vi "CSTK_Icon_Creator_Dialong_InputPath.vi"(0 "Enable":bool=TRUE caption="启用", 1 "分类文件夹名输入":string caption="分类文件夹名", 5 "error in (no error)":errorcluster caption="错误输入（无错误）", 6 "名称":enum16{"分类文件夹名", "LOGO文件夹名"}(ring)) -> (17 "分类文件夹名输出":string caption="分类文件夹名", 18 "确定":bool, 19 "error out":errorcluster caption="错误输出")   [LabVIEW 2015, in "CSTK_Icon Creator.lvlib"]
doc: "显示标准对话框，提示用户输入用户名、密码等信息。\n--------------------\n\n该Express VI配置如下:\n\n显示给用户的信息:请输入分类文件夹名\n该输入为: \n文本输入框: 分类文件夹名"
uses:
  CSTK_Icon Creator.lvlib
panel:
  in  "分类文件夹名":string
  in  "Cancel":bool caption="取消"
  in  "OK2":bool
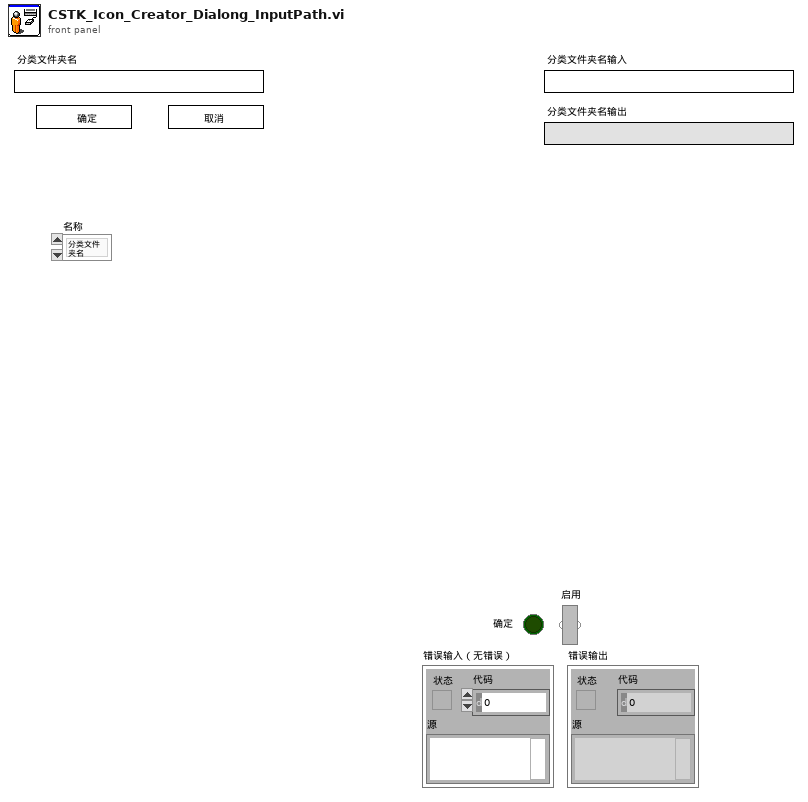
[diagram p1: front panel]
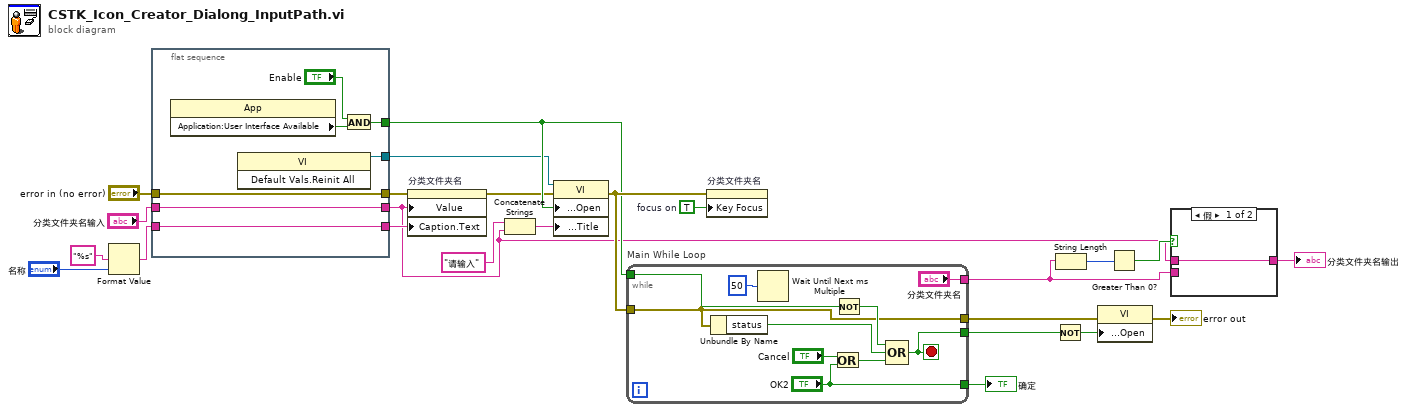
[diagram p0: block diagram]
diagram:
  w17 = TRUE  # focus on
  n1 = Format Value(format string="%s" ("格式字符串"), value (0)="名称") -> (output string=w5:string)  [unwired: 1 in]
  n2 = flat-sequence {
    tunnel: [w30] -> w19
    tunnel: [w28] -> w18
    tunnel: [w27] -> w14
    tunnel: "error in (no error)" -> [w27]
    tunnel: [w26] -> w2
    tunnel: "分类文件夹名输入" -> [w26]
    tunnel: w5 -> [w25]
    tunnel: [w25] -> w4
    frame #0 {
      n3 = property class="App"() -> ("Application:User Interface Available"=w29:bool)  [unwired: 2 in, 2 out]
      n4 = invoke class="VI" method="Default Vals.Reinit All"() -> (reference out=w28:refnum<vi>)  [unwired: 3 in, 2 out]
      n5 = And(x="Enable", y=w29) -> (x .and. y?=w30:bool)
    }
  }
  n6 = property on="分类文件夹名" class="Str"(error in=w14, "Value"=w2, "Caption.Text"=w4) -> (error out=w13:errorcluster)  [unwired: 1 in, 1 out]
  n7 = Concatenate Strings("请输入" ("字符串"), w2) -> (w1:string)
  n8 = property class="VI"(reference=w18, error in=w13, "Front Panel Window:Open"=w19, "Front Panel.Title"=w1) -> (error out=w22:errorcluster)  [unwired: 1 out]
  n9 = while "Main While Loop" {
    tunnel: ["OK2"] -> w12
    tunnel: w19 -> [w39]
    tunnel: [w37] -> w23
    tunnel: w22 -> [w36]
    tunnel: [w36] -> w21
    tunnel: ["分类文件夹名"] -> w8
    stop <- w37 stop-if-true
    n10 = Unbundle By Name(w36) -> ("status"=w34:bool)
    n11 = Wait Until Next ms Multiple(millisecond multiple=u32 50) -> ()  [unwired: 1 out]
    n12 = Or(x="Cancel", y="OK2") -> (x .or. y?=w35:bool)
    n13 = Not(x=w39) -> (.not. x?=w38:bool)
    n14 = Compound Arithmetic op=OR(w38, w34, w35) -> (w37:bool)
  }
  "确定" <- w12
  n15 = property on="分类文件夹名" class="Str"(error in=w22, "Key Focus"=w17) -> ()  [unwired: 1 in, 2 out]
  n16 = Not(x=w23) -> (.not. x?=w24:bool)
  n17 = String Length(string=w8) -> (length=w11:i32)
  n18 = property class="VI"(error in=w21, "Front Panel Window:Open"=w24) -> (error out=→"error out":errorcluster)  [unwired: 1 in, 1 out]
  n19 = Greater Than 0?(x=w11) -> (x > 0?=w10:bool)
  n20 = case shown="假" w10 {
    tunnel: [w42 w43] -> w9
    tunnel: w8 -> [_ w43]
    tunnel: w2 -> [w42 _]
    frame False {
    }
    frame True {
    }
  }
  "分类文件夹名输出" <- w9
